vi "SetText.vi"(8 "error in (no error)":errorcluster, 10 "Text":string, 11 "Markdown in":refnum<class "Markdown.lvclass">) -> (0 "error out":errorcluster, 3 "Markdown out":refnum<class "Markdown.lvclass">)   [LabVIEW 2021, in "LvMarkdown.lvlib" / "Markdown.lvclass"]
uses:
  Markdown.lvclass
  Markdown.lvclass/Markdown.ctl
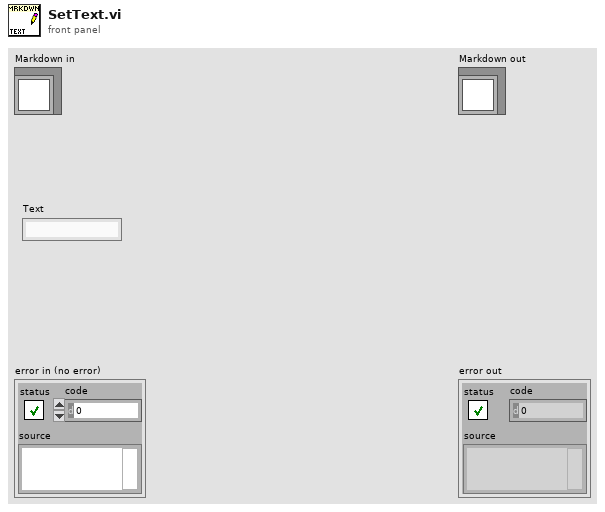
[diagram p1: front panel]
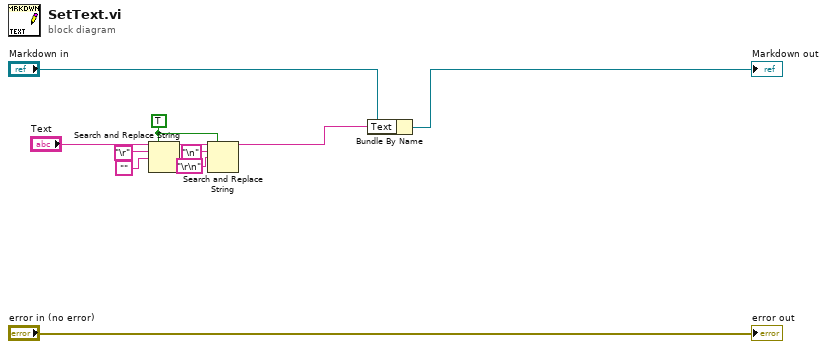
[diagram p0: block diagram]
diagram:
  w1 = TRUE ("replace all? (F)")
  n1 = Search and Replace String(replace all?=w1, input string="Text", search string="\r", replace string="") -> (result string=w5:string)  [unwired: 4 in, 3 out]
  n2 = Search and Replace String(replace all?=w1, input string=w5, search string="\n", replace string="\r\n") -> (result string=w4:string)  [unwired: 4 in, 3 out]
  n3 = Bundle By Name(cluster="Markdown in", "Text"=w4) -> (→"Markdown out":refnum<class "Markdown.lvclass">)
  "error out" <- "error in (no error)"
